vi "绘图-分段颜色-单环.vi"(7 "分段颜色":enum32{"蓝色", "红色"}(ring), 8 "基准索引":i32, 9 "光谱值":dbl, 11 "清空":bool) -> (3 "数组":dbl[][](array[numeric]))   [LabVIEW 2026, in "UI-无创.lvlib"]
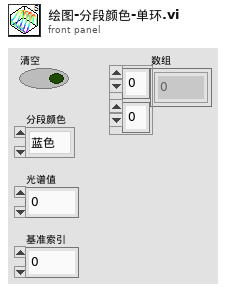
[diagram p1: front panel]
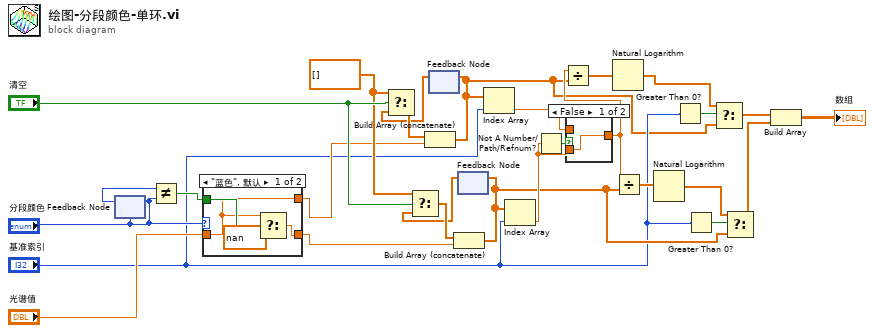
[diagram p0: block diagram]
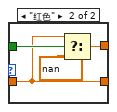
[diagram p2: hidden frame]
diagram:
  w18 = dbl[] []
  n1 = feedback #1("分段颜色") -> (w17:enum32{"蓝色", "红色"})
  n2 = feedback-in #1("分段颜色") -> ()
  n3 = Not Equal?(x=w17, y="分段颜色") -> (x != y?=w16:bool)
  n4 = case shown="\"蓝色\", 默认" "分段颜色" {
    tunnel: "光谱值" -> [w29 w35]
    tunnel: [w29 w33] -> w15
    tunnel: [w30 w35] -> w14
    tunnel: w16 -> [w32 w36]
    frame "蓝色", Default {
      n5 = Select(t=w29, s=w32, f=nan) -> (s? t:f=w30:dbl)
    }
    frame "红色" {
      n6 = Select(t=w35, s=w36, f=nan) -> (s? t:f=w33:dbl)
    }
  }
  n7 = feedback #2() -> (w19:dbl[])  [unwired: 1 in]
  n8 = Select(t=w18, s="清空", f=w19) -> (s? t:f=w20:dbl[])
  n9 = Build Array (concatenate)(w20, w15) -> (w2:dbl[])
  n10 = feedback-in #2(w2) -> ()
  n11 = feedback #3() -> (w21:dbl[])  [unwired: 1 in]
  n12 = Select(t=w18, s="清空", f=w21) -> (s? t:f=w22:dbl[])
  n13 = Build Array (concatenate)(w22, w14) -> (w7:dbl[])
  n14 = feedback-in #3(w7) -> ()
  n15 = Index Array(array=w2, index="基准索引") -> (element=w26:dbl)
  n16 = Index Array(array=w7, index="基准索引") -> (element=w27:dbl)
  n17 = Not A Number/Path/Refnum?(number/path/refnum=w27) -> (NaN/Path/Refnum?=w25:bool)
  n18 = case shown="False" w25 {
    tunnel: w26 -> [_ w38]
    tunnel: w27 -> [w37 _]
    tunnel: [w37 w38] -> w28
    frame False {
    }
    frame True {
    }
  }
  n19 = Divide(x=w28, y=w2) -> (x/y=w11:dbl[])
  n20 = Natural Logarithm(1:w11) -> (0:w3:dbl[])
  n21 = Divide(x=w28, y=w7) -> (x/y=w10:dbl[])
  n22 = Natural Logarithm(1:w10) -> (0:w8:dbl[])
  n23 = Greater Than 0?(x="基准索引") -> (x > 0?=w5:bool)
  n24 = Greater Than 0?(x="基准索引") -> (x > 0?=w9:bool)
  n25 = Select(t=w3, s=w5, f=w2) -> (s? t:f=w1:dbl[])
  n26 = Select(t=w8, s=w9, f=w7) -> (s? t:f=w6:dbl[])
  n27 = Build Array(w1, w6) -> (→"数组":dbl[][])
